vi "init.vi"(8 "error in":errorcluster, 10 "TBM module configuration in":refnum<class "TBM module configuration.lvclass">, 11 "OPC UA runtime in":refnum<class "OPC UA Client runtime.lvclass">) -> (0 "error out":errorcluster, 1 "data allocations":T1, 2 "execution settings":T4, 3 "OPC UA runtime out":refnum<class "OPC UA Client runtime.lvclass">)   [LabVIEW 2014, in "OPC UA Client runtime.lvclass"]
doc: "Provides an interface for initializing a module at runtime. While this interface performs no operations, a child should provide an override which may open any necessary references or sessions, allocate necessary memory, and perform any final configuration validataion before providing the full configuration <b>execution data</b> to the calling process."
uses:
  OPC UA Client runtime.lvclass
  <vilib>/NI/Tag Bus Module Framework/module configuration/TBM module configuration.lvclass
  <vilib>/NI/Tag Bus Module Framework/runtime/execution settings.ctl
  <vilib>/NI/Tag Bus Module Framework/channel/data tables.ctl
  <vilib>/NI/Tag Bus/dictionary/data dictionary.lvclass
  <vilib>/NI/Tag Bus/dictionary table pair.ctl
  <vilib>/NI/Tag Bus/table/data table.ctl
  configuration/OPC UA Client configuration.lvclass
  configuration/OPC UA Client configuration.lvclass/OPC UA Client configuration.ctl
  <vilib>/NI/Tag Bus Module Framework/channel/TBM channel.lvclass/TBM channel.ctl
  OPC UA Client runtime.lvclass/OPC UA Client runtime.ctl
  <vilib>/NI/Tag Bus/tag/Data Type.ctl
  configuration/OPC UA Data Type.ctl
  <vilib>/NI/Tag Bus/tag/tag descriptor.lvclass/tag descriptor.ctl
  <vilib>/NI/Tag Bus Module Framework/channel/TBM channel.lvclass
  <vilib>/NI/Tag Bus Module Framework/runtime/TBM module execution interface.lvclass
  <vilib>/NI/Tag Bus/tag/tag descriptor.lvclass
  <vilib>/NI/Tag Bus/tag bus.lvlib
  <vilib>/NI/Tag Bus/table/data table.lvlib
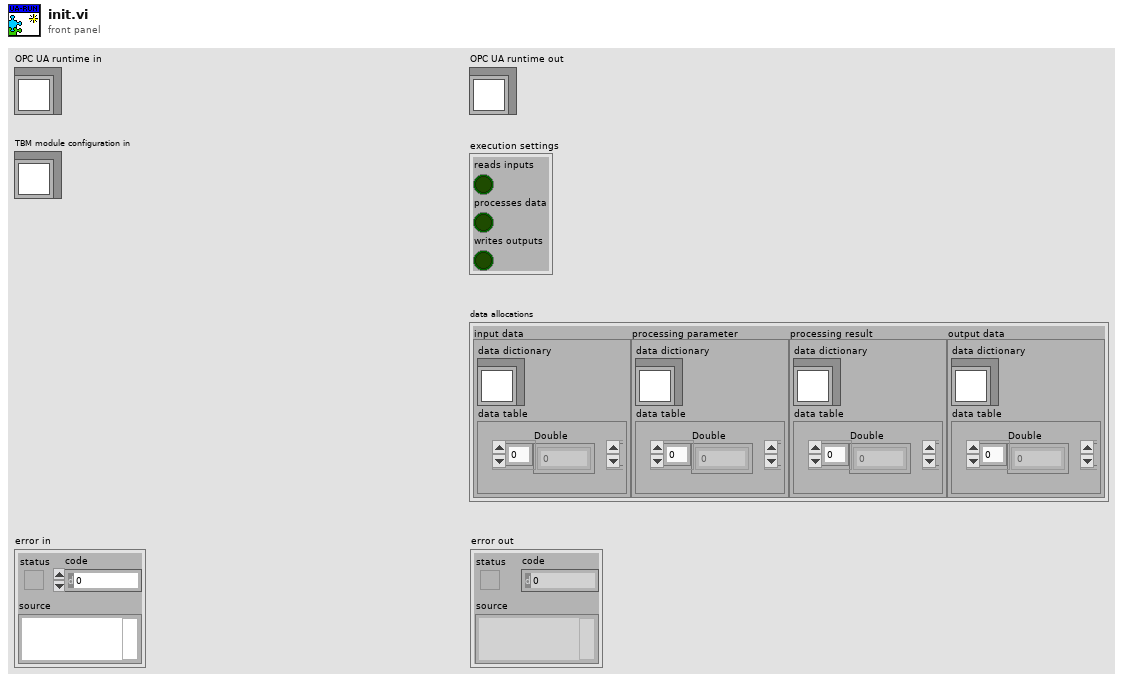
[diagram p1: front panel]
types:
  T1 = typedef "TBM channel.lvclass/data tables.ctl" = cluster{"input data":T2, "processing parameter":T2, "processing result":T2, "output data":T2}
  T2 = typedef "tag bus.lvlib/dictionary table pair.ctl" = cluster{"data dictionary":refnum<class "data dictionary.lvclass">, "data table":T3}
  T3 = typedef "tag bus.lvlib/data table.lvlib/data table.ctl" = cluster{"Double":dbl[], "Single":sgl[], "I64":i64[], "I32":i32[], "I16":i16[], "I8":i8[], "U64":u64[], "U32":u32[], "U16":u16[], "U8":u8[], "Boolean":bool[], "String":string[], "Array of Double":cluster{"DBL Array":dbl[]}[], "Array of Single":cluster{"SGL Array":sgl[]}[], "Array of I64":cluster{"I64 Array":i64[]}[], "Array of I32":cluster{"I32 Array":i32[]}[], "Array of I16":cluster{"I16 Array":i16[]}[], "Array of I8":cluster{"I8 Array":i8[]}[], "Array of U64":cluster{"U64 Array":u64[]}[], "Array of U32":cluster{"U32 Array":u32[]}[], "Array of U16":cluster{"U16 Array":u16[]}[], "Array of U8":cluster{"U8 Array":u8[]}[], "Array of Boolean":cluster{"Boolean Array":bool[]}[], "Array of String":cluster{"String Array":string[]}[]}
  T4 = typedef "TBM module execution interface.lvclass/execution settings.ctl" = cluster{"reads inputs":bool, "processes data":bool, "writes outputs":bool}
  T5 = typedef "tag bus.lvlib/tag descriptor.lvclass/Data Type.ctl" = enum16{"Double", "Single", "I64", "I32", "I16", "I8", "U64", "U32", "U16", "U8", "Boolean", "String", "Array of Double", "Array of Single", "Array of I64", "Array of I32", "Array of I16", "Array of I8", "Array of U64", "Array of U32", "Array of U16", "Array of U8", "Array of Boolean", "Array of String"}
  T6 = typedef "OPC UA Client configuration.lvclass/OPC UA Data Type.ctl" = u16
  T7 = cluster{"DCAF Data Type":T5, "Index":i32, "Node Path":string, "OPC UA Data Type":T6}
  T8 = typedef "OPC UA Client configuration.lvclass/Line.ctl" = cluster{"channel":refnum<class "TBM channel.lvclass">, "Node Path":string, "OPC UA Data Type":T6}
  T9 = typedef "TBM channel.lvclass/channel classification.ctl" = enum16{"input data", "output data", "processing parameter", "processing result"}
  T10 = cluster{"DCAF Data Type":T5, "Index":i32, "Node Path":string, "OPC UA Data Type":T6}[]
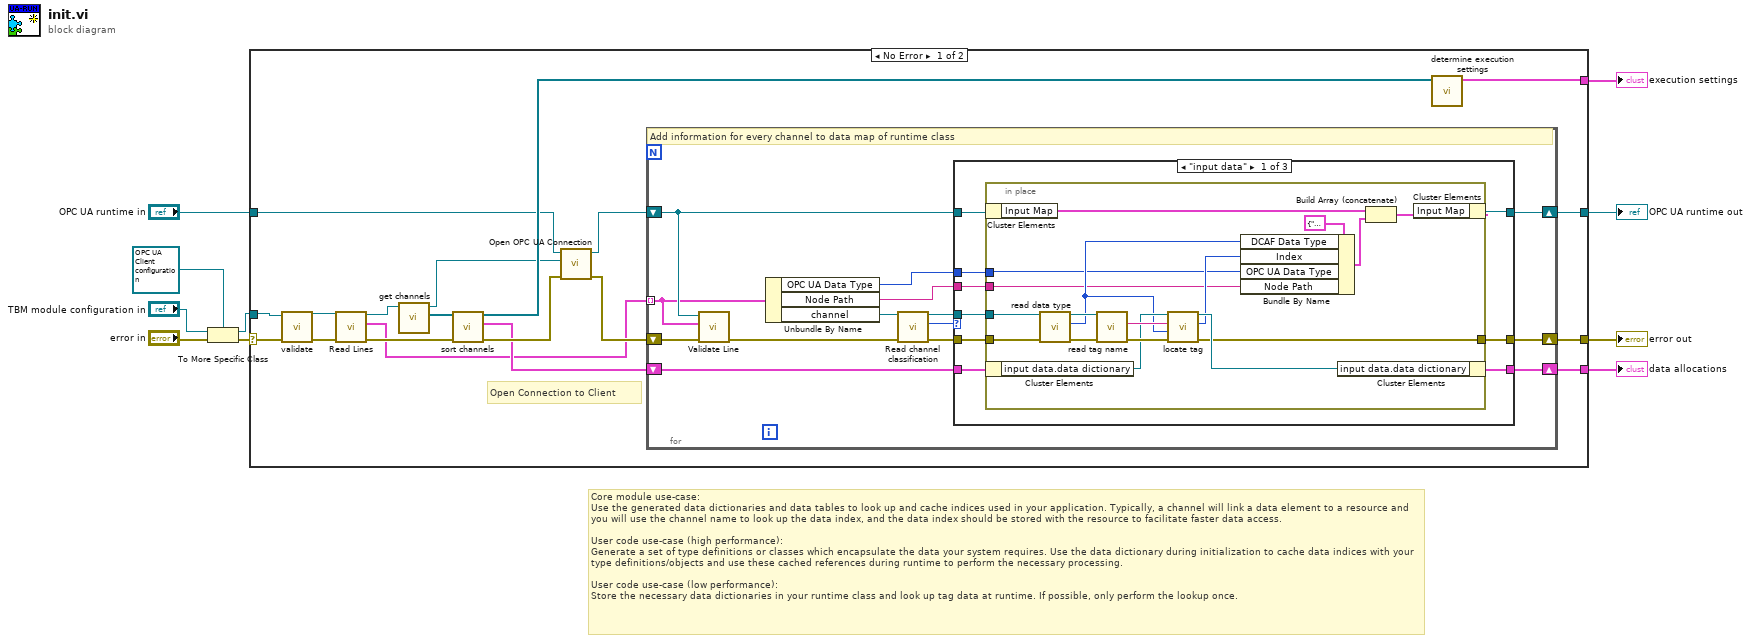
[diagram p0: block diagram]
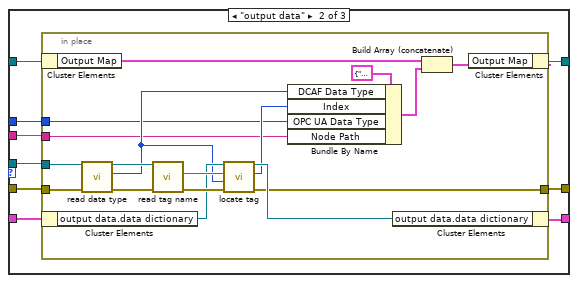
[diagram p2: hidden frame]
diagram:
  # "Core module use-case:\nUse the generated data dictionaries and data tables to look up and cache indices used in your application. Typically, a channel will link a data element to a resource and you will use the channel name to look up the data index, and the data index should be stored with the resource to facilitate faster data access.\n\nUser code use-case (high performance):\nGenerate a set of type definitions or classes which encapsulate the data your system requires. Use the data dictionary during initialization to cache data indices with your type definitions/objects and use these cached references during runtime to perform the necessary processing.\n\nUser code use-case (low performance):\nStore the necessary data dictionaries in your runtime class and look up tag data at runtime. If possible, only perform the lookup once."
  n1 = To More Specific Class(target class=refnum<class "OPC UA Client configuration.lvclass"> refnum ("Synchronous module configuration"), reference="TBM module configuration in", error in="error in") -> (specific class reference=w9:refnum<class "OPC UA Client configuration.lvclass">, error out=w10:errorcluster)
  n2 = case shown="No Error" w10 {
    selector: w10 -> [w28 w99]
    tunnel: w9 -> [w27 _]
    tunnel: "OPC UA runtime in" -> [w11 w100]
    tunnel: [w15 w100] -> w6
    tunnel: [w20 w99] -> w5
    tunnel: [w29 _] -> w4
    tunnel: [w14 _] -> w2
    frame No Error {
      # "Open Connection to Client"
      n3 = call-dynamic "validate.vi"("error in"=w28, "OPC UA configuration in"=w27) -> ("error out"=w18:errorcluster, "OPC UA configuration out"=w13:refnum<class "OPC UA Client configuration.lvclass">)  [unwired: 8 in]
      n4 = call "Read Lines.vi"("error in (no error)"=w18, "OPC UA configuration in"=w13) -> ("error out"=w17:errorcluster, "Lines"=w16:T8[], "OPC UA configuration out"=w19:refnum<class "OPC UA Client configuration.lvclass">)  [unwired: 7 in]
      n5 = call-dynamic "get channels.vi"("OPC UA configuration in"=w19) -> ("channels"=w26:refnum<class "TBM channel.lvclass">[], "OPC UA configuration out"=w12:refnum<class "OPC UA Client configuration.lvclass">)  [unwired: 9 in]
      n6 = call <vilib>:"sort channels.vi"("error in"=w17, "channels in"=w26) -> ("error out"=w25:errorcluster, "data allocations"=w21:T1, "channels out"=w22:refnum<class "TBM channel.lvclass">[])  [unwired: 7 in]
      n7 = call "Open OPC UA Connection.vi"("error in (no error)"=w25, "OPC UA configuration"=w12, "OPC UA runtime in"=w11) -> ("error out"=w24:errorcluster, "OPC UA runtime out"=w23:refnum<class "OPC UA Client runtime.lvclass">)  [unwired: 7 in]
      n8 = for {
        shift-right: [w39] -> w20
        shift-left: w24 -> [w33]
        shift-right: [w40] -> w15
        shift-left: w23 -> [w31]
        shift-right: [w37] -> w14
        shift-left: w21 -> [w38]
        tunnel: w16 -> [w30] mode=indexing
        # "Add information for every channel to data map of runtime class"
        n9 = call "Validate Line.vi"("error in (no error)"=w33, "Line"=w30, "OPC UA runtime in"=w31) -> ("error out"=w32:errorcluster)  [unwired: 8 in]
        n10 = Unbundle By Name(w30) -> ("OPC UA Data Type"=w34:T6, "Node Path"=w35:string, "channel"=w36:refnum<class "TBM channel.lvclass">)
        n11 = call <vilib>:"Read channel classification.vi"("error in"=w32, "channel in"=w36) -> ("error out"=w41:errorcluster, "channel classification"=w43:T9, "channel out"=w42:refnum<class "TBM channel.lvclass">)  [unwired: 7 in]
        n12 = case shown="\"input data\"" w43 {
          tunnel: w42 -> [w49 w76 _]
          tunnel: w41 -> [w50 w75 w97]
          tunnel: [w46 w71 w98] -> w40
          tunnel: w31 -> [w52 w78 w98]
          tunnel: [w48 w72 w97] -> w39
          tunnel: w38 -> [w51 w74 w96]
          tunnel: [w47 w73 w96] -> w37
          tunnel: w35 -> [w45 w77 _]
          tunnel: w34 -> [w44 w70 _]
          frame "input data" {
            n13 = in-place {
              in-place-border: w50 -> [w65]
              in-place-border: w49 -> [w67]
              in-place-border: [w57] -> w48
              in-place-border: w45 -> [w56]
              in-place-border: w44 -> [w53]
              n14 = in-place-cluster #1(w52) -> ("Input Map"=w68:T10)
              n15 = in-place-cluster #2(w51) -> ("input data.data dictionary"=w61:refnum<class "data dictionary.lvclass">)
              n16 = call <vilib>:"read data type.vi"("error in"=w65, "system tag in"=w67) -> ("error out"=w66:errorcluster, "data type"=w60:T5, "system tag out"=w62:refnum<class "TBM channel.lvclass">)  [unwired: 7 in]
              n17 = call <vilib>:"read tag name.vi"("error in"=w66, "system tag in"=w62) -> ("error out"=w64:errorcluster, "name"=w63:string)  [unwired: 7 in, 1 out]
              n18 = call <vilib>:"locate tag.vi"("error in"=w64, "data type"=w60, "name"=w63, "data dictionary in"=w61) -> ("error out"=w57:errorcluster, "index"=w58:i32, "data dictionary out"=w59:refnum<class "data dictionary.lvclass">)  [unwired: 5 in]
              n19 = Bundle By Name(cluster=T7 {"DCAF Data Type"=enum."Double", "Index"=0, "Node Path"="", "OPC UA Data Type"=0} ("Item"), "DCAF Data Type"=w60, "Index"=w58, "OPC UA Data Type"=w53, "Node Path"=w56) -> (w55:T7)
              n20 = in-place-cluster #2("input data.data dictionary"=w59) -> (w47:T1)
              n21 = Build Array (concatenate)(w68, w55) -> (w69:T10)
              n22 = in-place-cluster #1("Input Map"=w69) -> (w46:refnum<class "OPC UA Client runtime.lvclass">)
            }
          }
          frame "output data" {
            n23 = in-place {
              in-place-border: w75 -> [w91]
              in-place-border: w76 -> [w93]
              in-place-border: [w83] -> w72
              in-place-border: w77 -> [w81]
              in-place-border: w70 -> [w80]
              n24 = in-place-cluster #3(w78) -> ("Output Map"=w94:T10)
              n25 = in-place-cluster #4(w74) -> ("output data.data dictionary"=w87:refnum<class "data dictionary.lvclass">)
              n26 = call <vilib>:"read data type.vi"("error in"=w91, "system tag in"=w93) -> ("error out"=w92:errorcluster, "data type"=w86:T5, "system tag out"=w88:refnum<class "TBM channel.lvclass">)  [unwired: 7 in]
              n27 = call <vilib>:"read tag name.vi"("error in"=w92, "system tag in"=w88) -> ("error out"=w90:errorcluster, "name"=w89:string)  [unwired: 7 in, 1 out]
              n28 = call <vilib>:"locate tag.vi"("error in"=w90, "data type"=w86, "name"=w89, "data dictionary in"=w87) -> ("error out"=w83:errorcluster, "index"=w84:i32, "data dictionary out"=w85:refnum<class "data dictionary.lvclass">)  [unwired: 5 in]
              n29 = Bundle By Name(cluster=T7 {"DCAF Data Type"=enum."Double", "Index"=0, "Node Path"="", "OPC UA Data Type"=0} ("Item"), "DCAF Data Type"=w86, "Index"=w84, "OPC UA Data Type"=w80, "Node Path"=w81) -> (w82:T7)
              n30 = in-place-cluster #4("output data.data dictionary"=w85) -> (w73:T1)
              n31 = Build Array (concatenate)(w94, w82) -> (w95:T10)
              n32 = in-place-cluster #3("Output Map"=w95) -> (w71:refnum<class "OPC UA Client runtime.lvclass">)
            }
          }
          frame Default {
          }
        }
      }
      n33 = call <vilib>:"determine execution settings.vi"("channels"=w22) -> ("execution settings"=w29:T4)  [unwired: 10 in]
    }
    frame Error {
    }
  }
  "error out" <- w5
  "OPC UA runtime out" <- w6
  "execution settings" <- w4
  "data allocations" <- w2
